vi "Test Owner Retires When Idle.vi"(8 "error in":errorcluster) -> (0 "error out":errorcluster)   [LabVIEW 2019, in "RemoteControl.ZMQ.Tests.lvclass"]
uses:
  RemoteControl.ZMQ.Tests.lvclass
  src/ZMQ.ContextManager/ZMQ.ContextManager.lvlib
  <userlib>/LevyLab/RemoteControl/RemoteControl/RemoteControl.lvclass
  C:/Users/patrick/Documents/GitHub/Instrument-Subsystems/RemoteControl.ZMQ/src/RemoteControl.ZMQ/RemoteControl.ZMQ.lvclass
  C:/Program Files/National Instruments/LabVIEW 2019/user.lib/LevyLab/RemoteControl/RemoteControl/RemoteControl.lvclass
  C:/Program Files/National Instruments/LabVIEW 2019/vi.lib/JKI/JKI SMO/SMO/SMO.lvclass
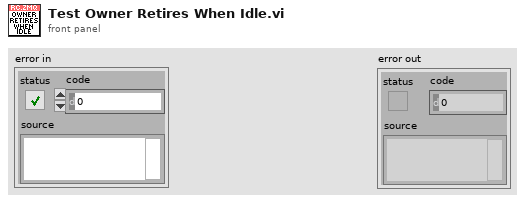
[diagram p1: front panel]
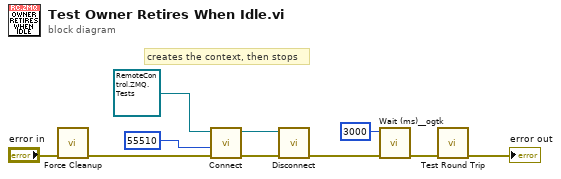
[diagram p0: block diagram]
diagram:
  # "creates the context, then stops"
  n1 = call "Force Cleanup.vi"("error in"="error in") -> ("error out"=w10:errorcluster)  [unwired: 9 in, 1 out]
  n2 = call <userlib>:"Connect.vi"("error in (no error)"=w10, "Port"=u16 55510, "RemoteControl in"=refnum<class "RemoteControl.ZMQ.Tests.lvclass"> refnum ("RemoteControl.ZMQ.Tests.lvclass")) -> ("error out"=w4:errorcluster, "RemoteControl out"=w2:refnum<class "RemoteControl.ZMQ.Tests.lvclass">)  [unwired: 7 in]
  n3 = call <userlib>:"Disconnect.vi"("error in (no error)"=w4, "RemoteControl in"=w2) -> ("error out"=w9:errorcluster)  [unwired: 8 in, 1 out]
  n4 = call <userlib>:"Wait (ms)__ogtk.vi"("error in (no error)"=w9, "milliseconds to wait"=u32 3000) -> ("error out"=w7:errorcluster)  [unwired: 8 in, 1 out]
  n5 = call "Test Round Trip.vi"("error in (no error)"=w7) -> ("error out"=→"error out":errorcluster)  [unwired: 10 in]
